vi "DAC Configure.vi"(8 "error in":errorcluster, 11 "DAC Inclino in":refnum<class "DAC Inclinometer.lvclass">) -> (0 "error out":errorcluster, 3 "DAC Inclino out":refnum<class "DAC Inclinometer.lvclass">)   [LabVIEW 2019, in "DAC.lvlib" / "DAC Inclinometer.lvclass"]
uses:
  DAC Inclinometer.lvclass
  C:/Users/wg/Documents/LV_Projects/test-stand/App/DAC/DAC.lvclass
  DAC.lvclass/DAC.ctl
  DAC Inclinometer.lvclass/DAC Inclinometer.ctl
  <vilib>/DAQmx/create/channels.llb/DAQmx Create Channel (AI-Voltage-Basic).vi
  DAC.lvclass
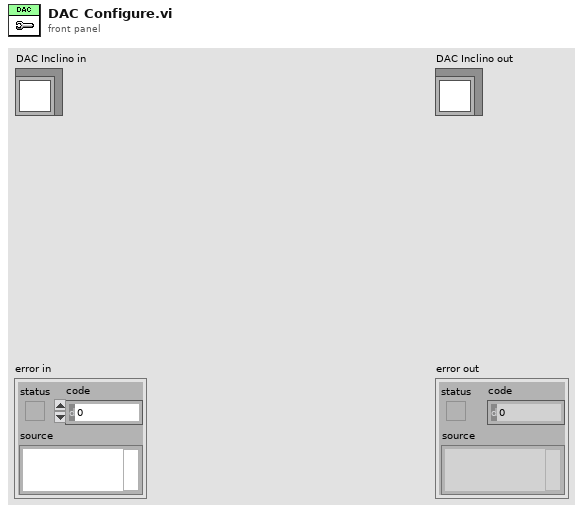
[diagram p1: front panel]
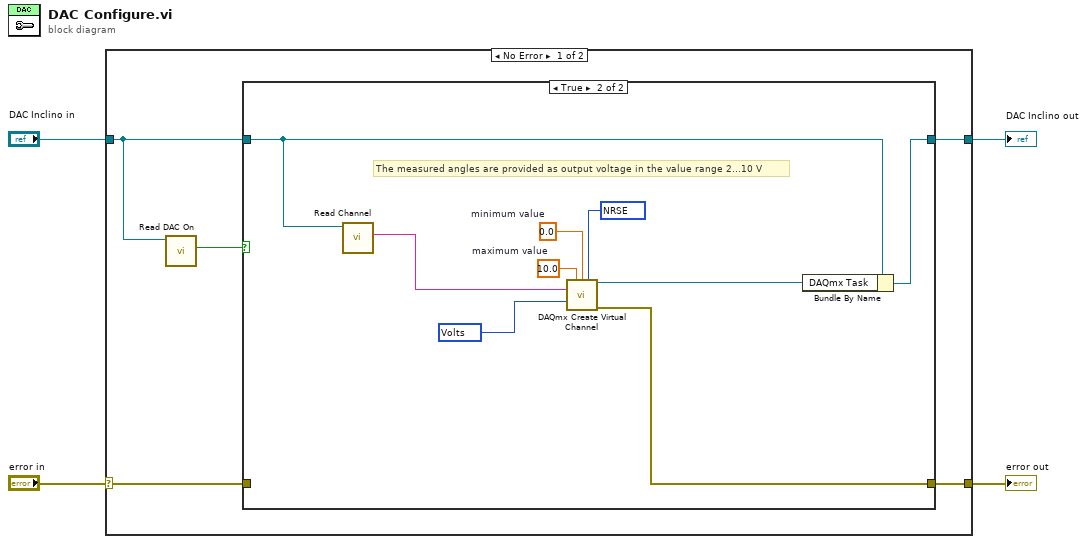
[diagram p0: block diagram]
diagram:
  n1 = case shown="No Error" "error in" {
    selector: "error in" -> [w6 w22]
    tunnel: [w5 w22] -> w4
    tunnel: [w7 w21] -> w3
    tunnel: "DAC Inclino in" -> [w9 w21]
    frame No Error {
      n2 = call "Read DAC On.vi"("DAC in"=w9) -> ("DAC On"=w8:bool)  [unwired: 8 in, 2 out]
      n3 = case shown="True" w8 {
        tunnel: w9 -> [w11 w13]
        tunnel: [w11 w20] -> w7
        tunnel: w6 -> [w10 _]
        tunnel: [w10 w18] -> w5
        frame False {
          # "Temperature measurement is off."
        }
        frame True {
          w14 = 10.0  # maximum value
          w15 = 0.0  # minimum value
          w16 = 10078 items=["Default"=-1, "RSE"=10083, "NRSE"=10078, "Differential"=10106, "Pseudodifferential"=12529] ("input terminal configuration")
          w17 = 10348 items=["Volts"=10348, "From Custom Scale"=10065] ("units")
          # "The measured angles are provided as output voltage in the value range 2...10 V"
          # "Temperature measurement is on."
          n4 = call "Read Channel.vi"("DAC in"=w13) -> ("Channel"=w12:string)  [unwired: 8 in, 2 out]
          n5 = call-poly <vilib>:"DAQmx Create Virtual Channel.vi"("maximum value"=w14, "minimum value"=w15, "input terminal configuration"=w16, "physical channels"=w12, "units"=w17) -> ("task out"=w19:refnum<k21>, "error out"=w18:errorcluster)  [unwired: 9 in]
          n6 = Bundle By Name(cluster=w13, "DAQmx Task"=w19) -> (w20:refnum<class "DAC Inclinometer.lvclass">)
        }
      }
    }
    frame Error {
    }
  }
  "error out" <- w4
  "DAC Inclino out" <- w3
